vi "Register Chart.vi"(8 "error in (no error)":errorcluster, 10 "Chart Registration":T1, 11 "Historian Charting Manager in":refnum<class "Historian Charting Manager.lvclass">) -> (0 "error out":errorcluster, 3 "Historian Charting Manager out":refnum<class "Historian Charting Manager.lvclass">)   [LabVIEW 2020, in "VolatusGUI.lvlib" / "Historian Charting Manager.lvclass"]
uses:
  Historian Charting Manager.lvclass
  Chart Registration.ctl
  Select Plot Group Data.ctl
  Plot Group Config.ctl
  X-Axis Type.ctl
  Plot Config.ctl
  Scale.ctl
  Historian Charting Manager.lvclass/Historian Charting Manager.ctl
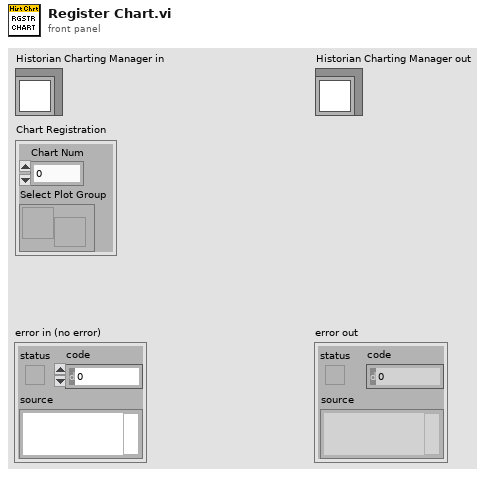
[diagram p1: front panel]
types:
  T1 = typedef "VolatusGUI.lvlib/Historian Charting Manager.lvclass/Chart Registration.ctl" = cluster{"Chart Num":i32, "Select Plot Group":refnum<user-event>}
  T2 = typedef "VolatusGUI.lvlib/Historian Charting Manager.lvclass/Plot Group Config.ctl" = cluster{"Name":string, "X-Axis Type":T3, "X-Axis Channel":string, "Plots":T4[], "Lock Now":bool, "Time":string, "Swap Axes":bool}
  T3 = typedef "VolatusGUI.lvlib/Historian Charting Manager.lvclass/X-Axis Type.ctl" = enum16{"Time", "Channel"}
  T4 = typedef "VolatusGUI.lvlib/Historian Charting Manager.lvclass/Plot Config.ctl" = cluster{"Channel":string, "Visible":bool, "Color":u32, "Scale":T5}
  T5 = typedef "VolatusGUI.lvlib/Historian Charting Manager.lvclass/Scale.ctl" = enum16{"Left", "Right"}
  T6 = typedef "VolatusGUI.lvlib/Historian Charting Manager.lvclass/Select Plot Group Data.ctl" = cluster{"Chart Num":i32, "Plots Config":T2, "Plot Groups":string[]}
  T7 = typedef "VolatusGUI.lvlib/Historian Charting Manager.lvclass/Chart Info.ctl" = cluster{"PluginGUI":refnum<class "MessageQ.lvclass">, "Select Plot Group":refnum<user-event>}
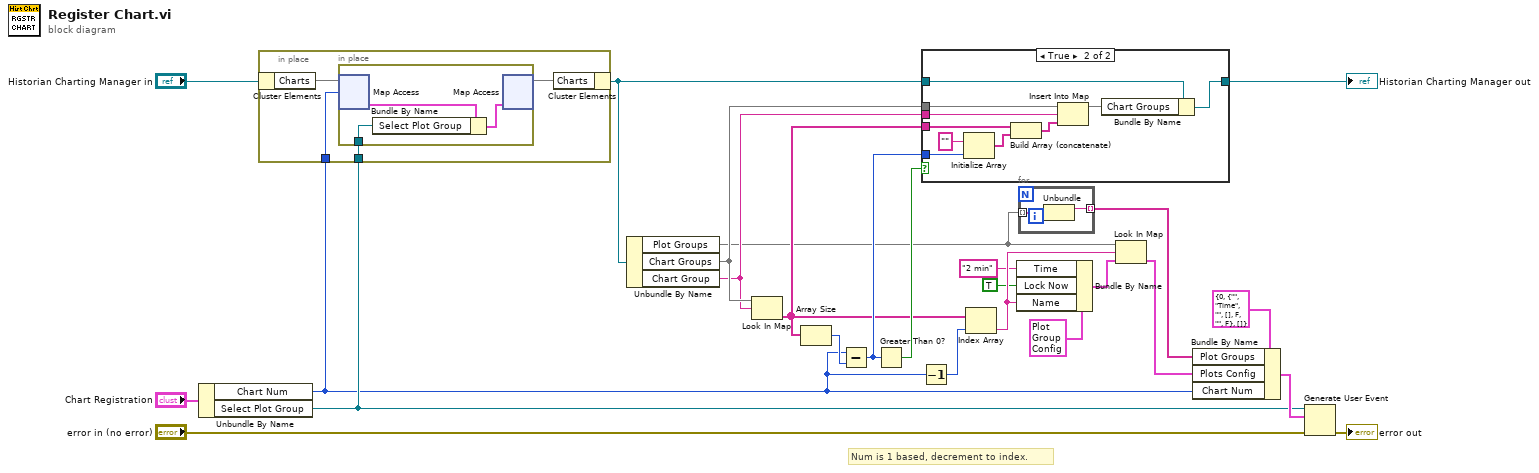
[diagram p0: block diagram]
diagram:
  # "Num is 1 based, decrement to index."
  n1 = Unbundle By Name("Chart Registration") -> ("Chart Num"=w3:i32, "Select Plot Group"=w19:refnum<user-event>)
  n2 = in-place {
    in-place-border: w3 -> [w28]
    in-place-border: w19 -> [w27]
    n3 = in-place-cluster #1("Historian Charting Manager in") -> ("Charts"=w29:map{i32, T7})
    n4 = in-place {
      in-place-border: w27 -> [w31]
      n5 = in-place-map #2(w29, w28) -> (w32:T7)  [unwired: 1 in, 1 out]
      n6 = Bundle By Name(cluster=w32, "Select Plot Group"=w31) -> (w30:T7)
      n7 = in-place-map #2(w30) -> (w26:map{i32, T7})  [unwired: 1 in, 2 out]
    }
    n8 = in-place-cluster #1("Charts"=w26) -> (w9:refnum<class "Historian Charting Manager.lvclass">)
  }
  n9 = Unbundle By Name(w9) -> ("Plot Groups"=w2:map{string, T2}, "Chart Groups"=w6:map{string, string[]}, "Chart Group"=w5:string)
  n10 = Look In Map(map=w6, key=w5) -> (value=w7:string[])  [unwired: 1 in, 1 out]
  n11 = Array Size(array=w7) -> (size(s)=w11:i32)
  n12 = Subtract(x=w3, y=w11) -> (x-y=w8:i32)
  n13 = Greater Than 0?(x=w8) -> (x > 0?=w10:bool)
  n14 = Decrement(x=w3) -> (x-1=w18:i32)
  n15 = case shown="True" w10 {
    tunnel: w9 -> [w33 w36]
    tunnel: w8 -> [_ w43]
    tunnel: w7 -> [_ w41]
    tunnel: w6 -> [_ w39]
    tunnel: w5 -> [_ w37]
    tunnel: [w33 w34] -> w4
    frame False {
    }
    frame True {
      n16 = Initialize Array("", w43) -> (w40:string[])
      n17 = Build Array (concatenate)(w41, w40) -> (w38:string[])
      n18 = Insert Into Map(map in=w39, key=w37, value=w38) -> (map out=w35:map{string, string[]})  [unwired: 2 out]
      n19 = Bundle By Name(cluster=w36, "Chart Groups"=w35) -> (w34:refnum<class "Historian Charting Manager.lvclass">)
    }
  }
  "Historian Charting Manager out" <- w4
  n20 = Index Array(array=w7, index=w18) -> (element=w14:string)
  n21 = Bundle By Name(cluster=T2 {"Name"="", "X-Axis Type"=enum."Time", "X-Axis Channel"="", "Plots"=[], "Lock Now"=TRUE, "Time"="2 min", "Swap Axes"=FALSE} ("default value"), "Time"="2 min", "Lock Now"=TRUE, "Name"=w14) -> (w15:T2)
  n22 = for {
    tunnel: w2 -> [w45] mode=indexing
    tunnel: [w44] -> w1 mode=indexing
    n23 = Unbundle(w45) -> ("Name"=w44:string)  [unwired: 1 out]
  }
  n24 = Look In Map(map=w2, key=w14, default value=w15) -> (value=w23:T2)  [unwired: 1 out]
  n25 = Bundle By Name(cluster=T6 {"Chart Num"=0, "Plots Config"={"Name"="", "X-Axis Type"=enum."Time", "X-Axis Channel"="", "Plots"=[], "Lock Now"=FALSE, "Time"="", "Swap Axes"=FALSE}, "Plot Groups"=[]} ("event data"), "Plot Groups"=w1, "Plots Config"=w23, "Chart Num"=w3) -> (w24:T6)
  n26 = Generate User Event(user event=w19, event data cluster=w24, error in="error in (no error)") -> (error out=→"error out":errorcluster)  [unwired: 1 in, 1 out]
